vi "Add Task.vi"(7 "Project Store in":refnum<class "Project Store.lvclass">, 8 "error in (no error)":errorcluster, 10 "Name":string, 11 "Project ID":string) -> (0 "error out":errorcluster, 3 "Task":T1, 5 "Project Store out":refnum<class "Project Store.lvclass">)   [LabVIEW 2024, in "Project Store.lvclass"]
doc: "Adds a new task under the given project and returns its row. The task gets a new GUID as its ID, Active = TRUE, and Sort Order = the number of tasks that project already had, so it sorts last. The project ID is not checked. Nothing is written to disk until Write to Data Source.\n\nGenerated by: Claude"
uses:
  Project Store.lvclass
  Rows/Task.ctl
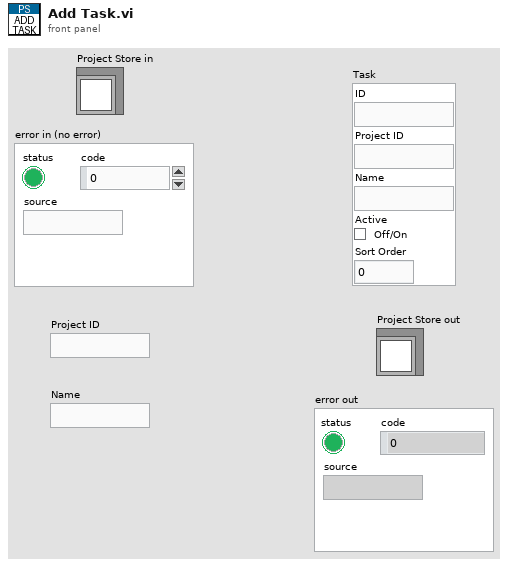
[diagram p1: front panel]
types:
  T1 = typedef "Task.ctl" = cluster{"ID":string, "Project ID":string, "Name":string, "Active":bool, "Sort Order":i32}
  T2 = typedef "Task List.ctl" = T1[]
  T3 = cluster{"NI GUID":string, "Project ID":string, "Name":string, "active":bool, i32}
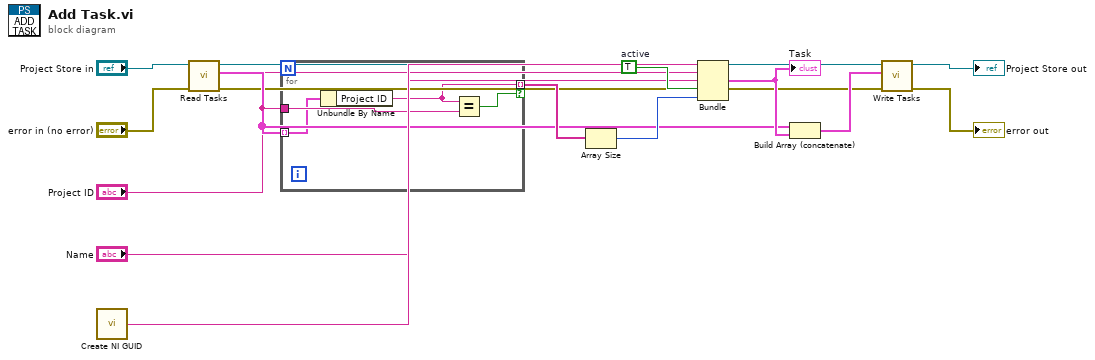
[diagram p0: block diagram]
diagram:
  w11 = TRUE  # active
  n1 = call <vilib>:"Create NI GUID.vi"() -> ("NI GUID"=w10:string)
  n2 = call-dynamic "Read Tasks.vi"("error in (no error)"="error in (no error)", "Project Store in"="Project Store in") -> ("error out"=w5:errorcluster, "Task List"=w7:T2, "Project Store out"=w6:refnum<class "Project Store.lvclass">)  [unwired: 7 in]
  n3 = for {
    tunnel: "Project ID" -> [w17]
    tunnel: w7 -> [w16] mode=indexing
    tunnel: [w18] -> w8 mode=indexing if=w19
    n4 = Unbundle By Name(w16) -> ("Project ID"=w18:string)
    n5 = Equal?(x=w18, y=w17) -> (x = y?=w19:bool)
  }
  n6 = Array Size(array=w8) -> (size(s)=w9:i32)
  n7 = Bundle("NI GUID"=w10, "Project ID"="Project ID", "Name"="Name", "active"=w11, w9) -> (w12:T3)  [unwired: 1 in]
  "Task" <- w12
  n8 = Build Array (concatenate)(w7, w12) -> (w13:T2)
  n9 = call-dynamic "Write Tasks.vi"("error in (no error)"=w5, "Task List"=w13, "Project Store in"=w6) -> ("error out"=→"error out":errorcluster, "Project Store out"=→"Project Store out":refnum<class "Project Store.lvclass">)  [unwired: 7 in]
